vi "pLogicEngine.vi"(7 "Update":bool, 8 "error in":errorcluster, 9 "Sequence":T3, 10 "data dictionary in":refnum<class "data dictionary.lvclass">, 11 "default data table":T2) -> (0 "error out":errorcluster, 2 "Rung":i32, 3 "data table out":T2)   [LabVIEW 2013]
uses:
  Controls/SequenceCluster.ctl
  <vilib>/NI/Tag Bus/table/data table.ctl
  <vilib>/NI/Tag Bus/dictionary/data dictionary.lvclass
  Controls/RungLogicState.ctl
  <vilib>/NI/Tag Bus/tag/Data Type.ctl
  <vilib>/NI/Tag Bus/table/data polymorphs/read one/read Boolean.vi
  <vilib>/NI/Tag Bus/table/data polymorphs/write one/write Boolean.vi
  <vilib>/NI/Tag Bus/tag/tag descriptor.lvclass
  <vilib>/NI/Tag Bus/table/data table.lvlib
panel:
  out "Array 2":T1[][](array[typedef])
  out "Array":string[][](array[string])
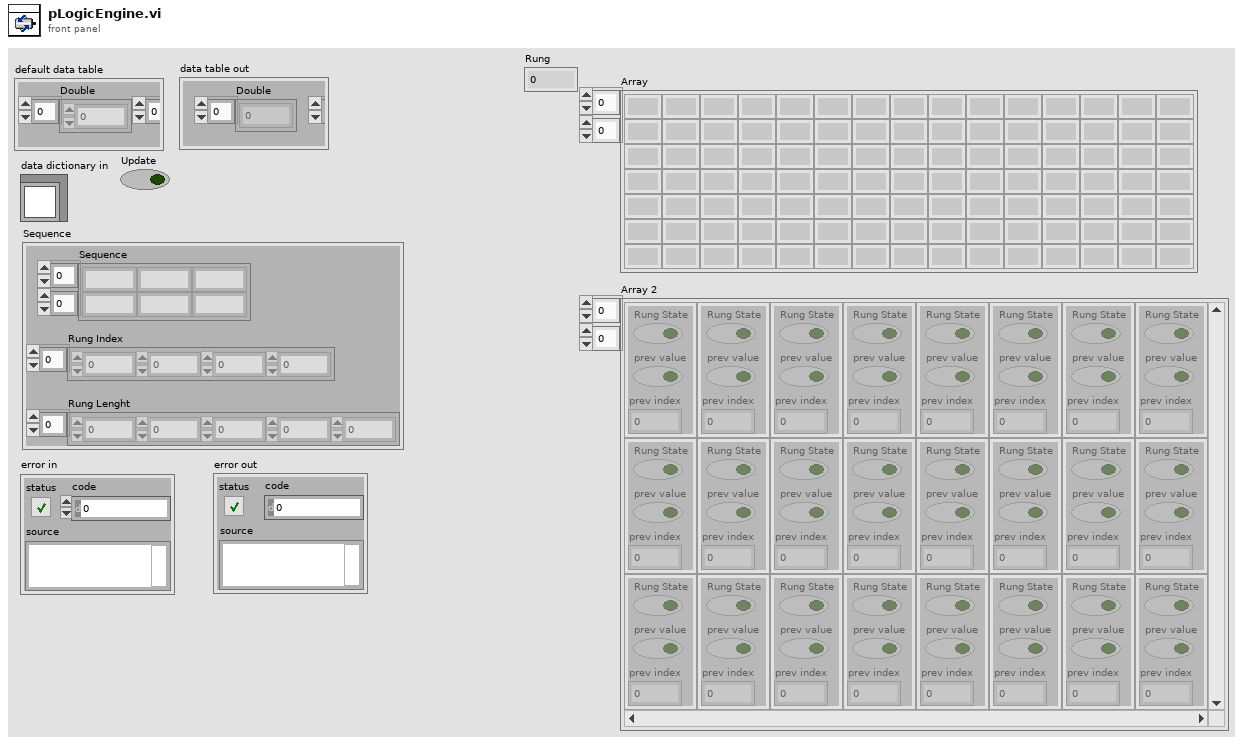
[diagram p1: front panel]
types:
  T1 = typedef "RungLogicState.ctl" = cluster{"Rung State":bool, "prev value":bool, "prev index":i32}
  T2 = typedef "tag bus.lvlib/data table.lvlib/data table.ctl" = cluster{"Double":dbl[], "Single":sgl[], "I64":i64[], "I32":i32[], "I16":i16[], "I8":i8[], "U64":u64[], "U32":u32[], "U16":u16[], "U8":u8[], "Boolean":bool[], "String":string[], "Array of Double":cluster{"DBL Array":dbl[]}[], "Array of Single":cluster{"SGL Array":sgl[]}[], "Array of I64":cluster{"I64 Array":i64[]}[], "Array of I32":cluster{"I32 Array":i32[]}[], "Array of I16":cluster{"I16 Array":i16[]}[], "Array of I8":cluster{"I8 Array":i8[]}[], "Array of U64":cluster{"U64 Array":u64[]}[], "Array of U32":cluster{"U32 Array":u32[]}[], "Array of U16":cluster{"U16 Array":u16[]}[], "Array of U8":cluster{"U8 Array":u8[]}[], "Array of Boolean":cluster{"Boolean Array":bool[]}[], "Array of String":cluster{"String Array":string[]}[]}
  T3 = typedef "SequenceCluster.ctl" = cluster{"Sequence":string[][], "Rung Index":i32[], "Rung Lenght":i32[]}
  T4 = typedef "tag bus.lvlib/tag descriptor.lvclass/Data Type.ctl" = enum16{"Double", "Single", "I64", "I32", "I16", "I8", "U64", "U32", "U16", "U8", "Boolean", "String", "Array of Double", "Array of Single", "Array of I64", "Array of I32", "Array of I16", "Array of I8", "Array of U64", "Array of U32", "Array of U16", "Array of U8", "Array of Boolean", "Array of String"}
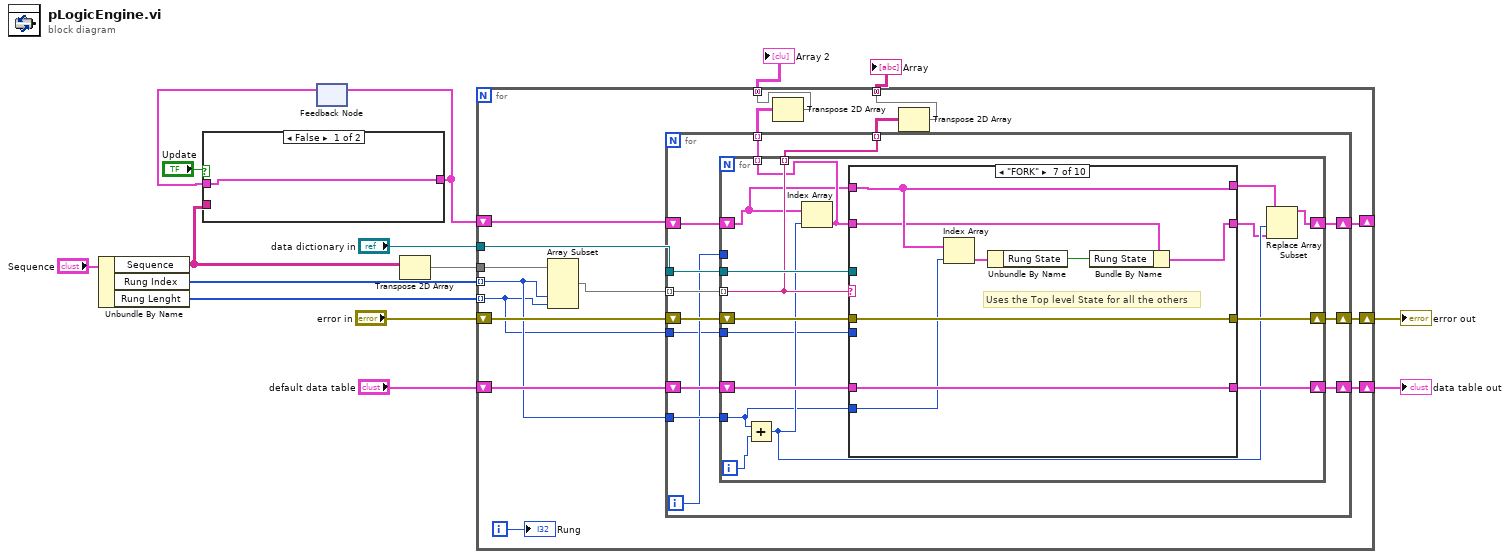
[diagram p0: block diagram]
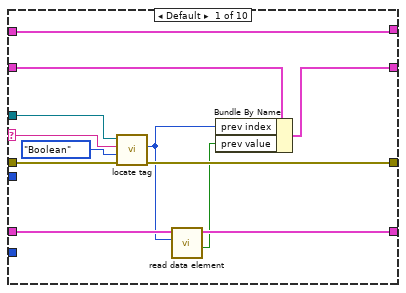
[diagram p2: hidden frame]
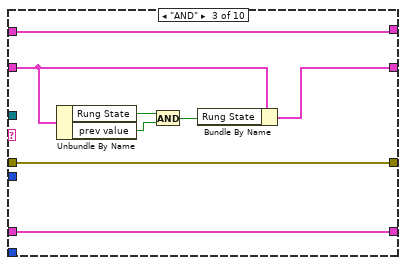
[diagram p4: hidden frame]
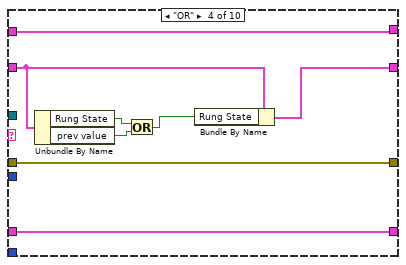
[diagram p5: hidden frame]
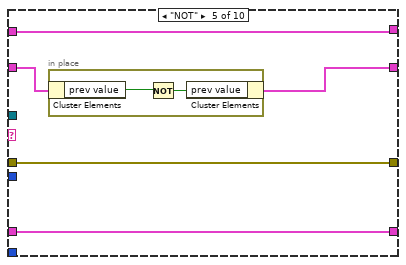
[diagram p6: hidden frame]
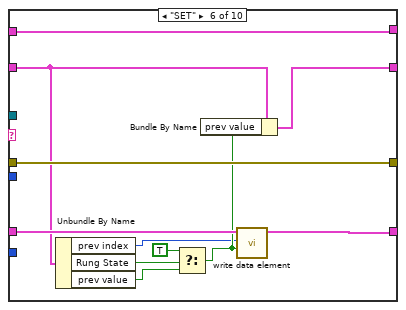
[diagram p7: hidden frame]
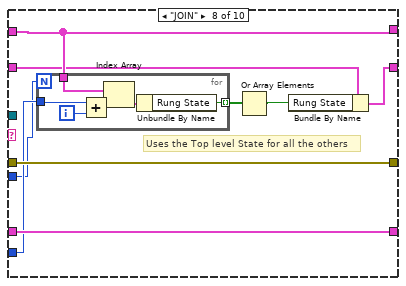
[diagram p8: hidden frame]
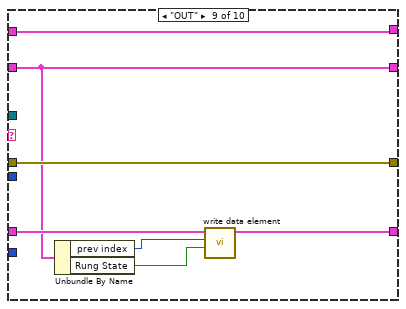
[diagram p9: hidden frame]
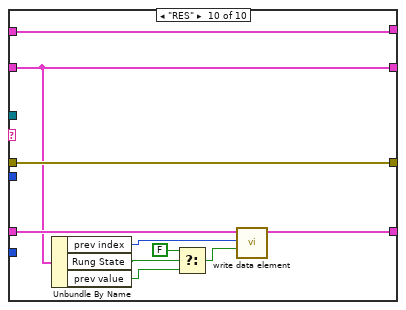
[diagram p10: hidden frame]
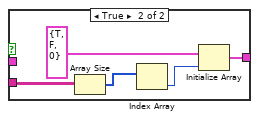
[diagram p11: hidden frame]
diagram:
  n1 = Unbundle By Name("Sequence") -> ("Sequence"=w3:string[][], "Rung Index"=w2:i32[], "Rung Lenght"=w1:i32[])
  n2 = feedback #1() -> (w7:T1[])  [unwired: 1 in]
  n3 = case shown="False" "Update" {
    tunnel: w3 -> [_ w21]
    tunnel: [w16 w17] -> w8
    tunnel: w7 -> [w16 _]
    frame False {
    }
    frame True {
      n4 = Array Size(array=w21) -> (size(s)=w19:i32[])
      n5 = Index Array(array=w19) -> (element=w18:i32)  [unwired: 1 in]
      n6 = Initialize Array(T1 {"Rung State"=TRUE, "prev value"=FALSE, "prev index"=0}, w18) -> (w17:T1[])
    }
  }
  n7 = feedback-in #1(w8) -> ()
  n8 = Transpose 2D Array(2D array=w3) -> (transposed array=w10:string[][])
  n9 = for {
    tunnel: "data dictionary in" -> [w36]
    tunnel: w10 -> [w31]
    tunnel: [w24] -> w6 mode=concatenating
    tunnel: [w26] -> w5 mode=concatenating
    shift-right: [w37] -> w15
    shift-left: "error in" -> [w34]
    shift-right: [w33] -> w4
    shift-left: "default data table" -> [w35]
    shift-right: [w32] -> _
    shift-left: w8 -> [w29]
    tunnel: w2 -> [w30] mode=indexing
    tunnel: w1 -> [w23] mode=indexing
    i -> [w22]
    n10 = Array Subset(array=w31, index (col)=w30, length (col)=w23) -> (w28:string[][])  [unwired: 2 in]
    n11 = for {
      tunnel: w28 -> [w50] mode=indexing
      tunnel: w36 -> [w47]
      shift-right: [w48] -> w33
      shift-left: w35 -> [w49]
      shift-right: [w45] -> w37
      shift-left: w34 -> [w46]
      tunnel: [w42] -> w25 mode=indexing
      tunnel: [w41] -> w27 mode=indexing
      tunnel: w30 -> [w40]
      shift-right: [w43] -> w32
      shift-left: w29 -> [w44]
      tunnel: w23 -> [w38]
      i -> [w39]
      n12 = for {
        tunnel: w50 -> [w60] mode=indexing
        tunnel: w47 -> [w65]
        shift-right: [w63] -> w48
        shift-left: w49 -> [w64]
        shift-right: [w61] -> w45
        shift-left: w46 -> [w62]
        tunnel: [w60] -> w42 mode=indexing
        tunnel: [w59] -> w41 mode=indexing
        tunnel: w40 -> [w52]
        shift-right: [w58] -> w43
        shift-left: w44 -> [w53]
        tunnel: w39 -> [_]
        tunnel: w38 -> [w51]
        i -> [w57]
        n13 = Add(x=w52, y=w57) -> (x+y=w56:i32)
        n14 = Index Array(array=w53, index=w56) -> (element=w59:T1)
        n15 = case shown="\"FORK\"" w60 {
          selector: w60 -> [w75 _ _ _ _ _ _ _ _ _]
          tunnel: w65 -> [w76 _ _ _ _ _ _ _ _ _]
          tunnel: w64 -> [w77 w81 w89 w97 w102 w114 w123 w132 w144 w152]
          tunnel: [w73 w81 w89 w97 w102 w106 w123 w132 w145 w155] -> w63
          tunnel: w62 -> [w72 w80 w88 w96 w101 w113 w122 w131 w143 w151]
          tunnel: [w71 w80 w88 w96 w101 w113 w122 w131 w143 w151] -> w61
          tunnel: [w67 w79 w86 w94 w99 w109 w117 w127 w142 w150] -> w55
          tunnel: w59 -> [w70 w79 w87 w95 w100 w110 w118 w128 w142 w150]
          tunnel: [w66 w78 w82 w90 w98 w105 w121 w130 w139 w146] -> w54
          tunnel: w53 -> [w66 w78 w82 w90 w98 w105 w121 w130 w139 w146]
          tunnel: w52 -> [_ _ _ _ _ _ w120 w129 _ _]
          tunnel: w51 -> [_ _ _ _ _ _ _ w124 _ _]
          frame Default {
            n16 = call <vilib>:"locate tag.vi"("error in"=w72, "data type"=Data_Type."Boolean", "name"=w75, "data dictionary in"=w76) -> ("error out"=w71:errorcluster, "index"=w69:i32)  [unwired: 5 in, 1 out]
            n17 = call-poly <vilib>:"read data element.vi"("index"=w69, "data table in"=w77) -> ("value"=w68:bool, "data table out"=w73:T2)  [unwired: 8 in]
            n18 = Bundle By Name(cluster=w70, "prev index"=w69, "prev value"=w68) -> (w67:T1)
          }
          frame "" {
          }
          frame "AND" {
            n19 = Unbundle By Name(w87) -> ("Rung State"=w84:bool, "prev value"=w83:bool)
            n20 = And(x=w84, y=w83) -> (x .and. y?=w85:bool)
            n21 = Bundle By Name(cluster=w87, "Rung State"=w85) -> (w86:T1)
          }
          frame "OR" {
            n22 = Unbundle By Name(w95) -> ("Rung State"=w93:bool, "prev value"=w92:bool)
            n23 = Or(x=w93, y=w92) -> (x .or. y?=w91:bool)
            n24 = Bundle By Name(cluster=w95, "Rung State"=w91) -> (w94:T1)
          }
          frame "NOT" {
            n25 = in-place {
              n26 = in-place-cluster #2(w100) -> ("prev value"=w104:bool)
              n27 = Not(x=w104) -> (.not. x?=w103:bool)
              n28 = in-place-cluster #2("prev value"=w103) -> (w99:T1)
            }
          }
          frame "SET" {
            n29 = Unbundle By Name(w110) -> ("prev index"=w107:i32, "Rung State"=w112:bool, "prev value"=w111:bool)
            n30 = Select(t=TRUE, s=w112, f=w111) -> (s? t:f=w108:bool)
            n31 = Bundle By Name(cluster=w110, "prev value"=w108) -> (w109:T1)
            n32 = call-poly <vilib>:"write data element.vi"("value"=w108, "index"=w107, "data table in"=w114) -> ("data table out"=w106:T2)  [unwired: 8 in]
          }
          frame "FORK" {
            # "Uses the Top level State for all the others"
            n33 = Index Array(array=w121, index=w120) -> (element=w119:T1)
            n34 = Unbundle By Name(w119) -> ("Rung State"=w116:bool)
            n35 = Bundle By Name(cluster=w118, "Rung State"=w116) -> (w117:T1)
          }
          frame "JOIN" {
            # "Uses the Top level State for all the others"
            n36 = for {
              N: w124 -> [_]
              tunnel: w130 -> [w138]
              tunnel: w129 -> [w134]
              tunnel: [w136] -> w126 mode=indexing
              i -> [w135]
              n37 = Add(x=w134, y=w135) -> (x+y=w133:i32)
              n38 = Index Array(array=w138, index=w133) -> (element=w137:T1)
              n39 = Unbundle By Name(w137) -> ("Rung State"=w136:bool)
            }
            n40 = Or Array Elements(Boolean array=w126) -> (logical OR=w125:bool)
            n41 = Bundle By Name(cluster=w128, "Rung State"=w125) -> (w127:T1)
          }
          frame "OUT" {
            n42 = Unbundle By Name(w142) -> ("prev index"=w140:i32, "Rung State"=w141:bool)
            n43 = call-poly <vilib>:"write data element.vi"("value"=w141, "index"=w140, "data table in"=w144) -> ("data table out"=w145:T2)  [unwired: 8 in]
          }
          frame "RES" {
            n44 = Unbundle By Name(w150) -> ("prev index"=w147:i32, "Rung State"=w148:bool, "prev value"=w149:bool)
            n45 = Select(t=FALSE, s=w148, f=w149) -> (s? t:f=w153:bool)
            n46 = call-poly <vilib>:"write data element.vi"("value"=w153, "index"=w147, "data table in"=w152) -> ("data table out"=w155:T2)  [unwired: 8 in]
          }
        }
        n47 = Replace Array Subset(array=w54, new element=w55, index=w56) -> (w58:T1[])
      }
    }
    n48 = Transpose 2D Array(2D array=w27) -> (transposed array=w26:T1[][])
    n49 = Transpose 2D Array(2D array=w25) -> (transposed array=w24:string[][])
    "Rung" <- w22
  }
  "error out" <- w15
  "data table out" <- w4
  "Array" <- w6
  "Array 2" <- w5
